vi "OpenG Empty Array template.vi"(2 "Array":dbl[](array[numeric])) -> (7 "Empty?":bool)   [LabVIEW 2012]
doc: "Returns TRUE if Array is empty (any dimension has length equal zero). Otherwise, this function returns FALSE.a"
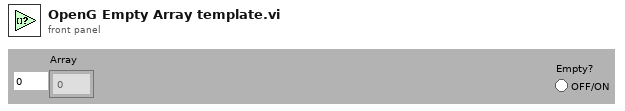
[diagram p1: front panel]
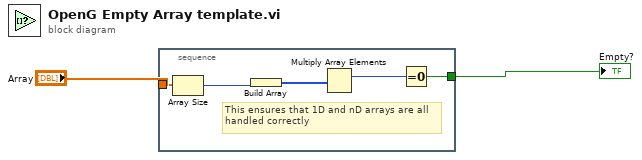
[diagram p0: block diagram]
diagram:
  n1 = stacked-sequence {
    tunnel: "Array" -> [w7]
    tunnel: [w3] -> w1
    frame #0 {
      # "This ensures that 1D and nD arrays are all\nhandled correctly"
      n2 = Array Size(array=w7) -> (size(s)=w6:i32)
      n3 = Build Array(w6) -> (w5:i32[])
      n4 = Multiply Array Elements(1:w5) -> (0:w4:i32)
      n5 = Equal To 0?(x=w4) -> (x = 0?=w3:bool)
    }
  }
  "Empty?" <- w1
